vi "AlliGator Phasor Plot Event Registration Refnums.vi"(8 "error in (no error)":errorcluster) -> (0 "error out":errorcluster, 2 "Phasor Plote Display Range Event":refnum<event-registration>, 3 "Phasor Plot Display Event":refnum<event-registration>)   [LabVIEW 2021, in "AlliGator Phasor Plot.lvlib"]
uses:
  AlliGator Phasor Plot.lvlib
panel:
  # "see the License on the block diagram (Ctrl+E or Window:Show Block Diagram)"
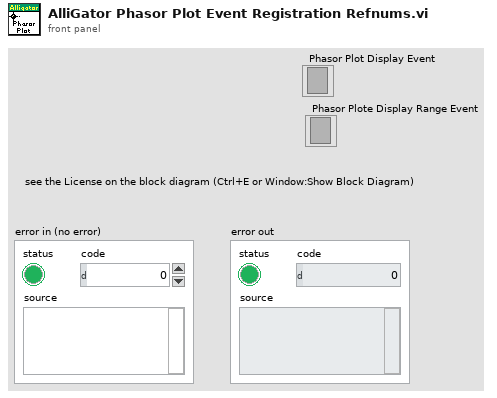
[diagram p1: front panel]
types:
  T1 = typedef "AlliGator Phasor Plot.lvlib/AlliGator Phasor Plot Ctrl Refnums.ctl" = cluster{"Phasor Ratio":refnum<vi>, "Modulus Lifetime":refnum<vi>, "Phasor at cursor (m, phi)":refnum<vi>, "Phase Lifetime":refnum<vi>, "Phasor at cursor (g, s)":refnum<vi>, "Phasor Plor Average Lifetime":refnum<vi>, "Phasor Plot Active":refnum<vi>, "Save Phasor Plot":refnum<vi>, "Image Overlay Color":refnum<vi>, "Phasor Plot Color Scale":refnum<vi>, "Reference 1 Button":refnum<vi>, "Reference 2 Button":refnum<vi>, "True Phasor Plot Value":refnum<vi>, "Phasor Plot Display Range":refnum<vi>, "Phasor Plot Display":refnum<vi>, "Phasor Plot Frequency":refnum<vi>, "Overlay Mode":refnum<vi>}
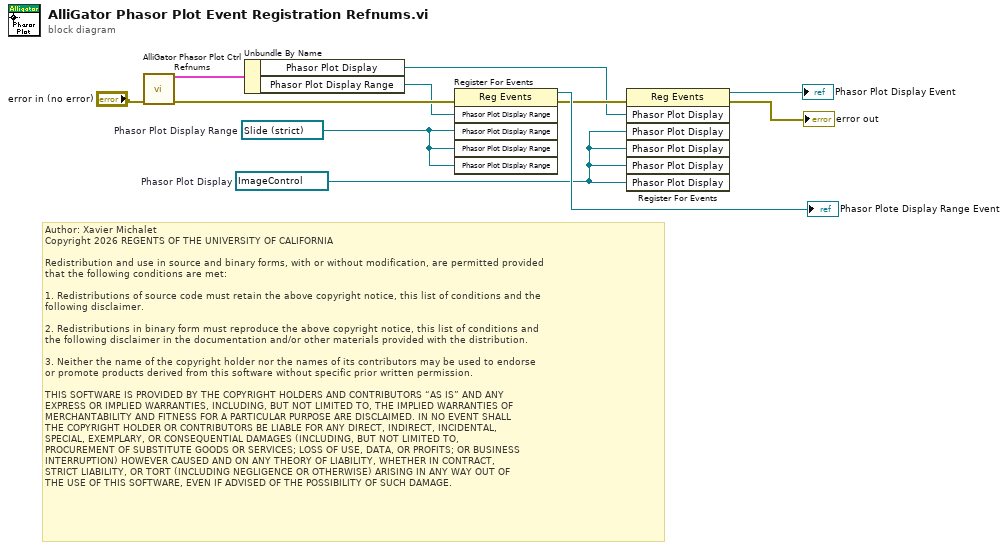
[diagram p0: block diagram]
diagram:
  w10 = refnum<vi> refnum  # Phasor Plot Display Range
  w1 = refnum<vi> refnum  # Phasor Plot Display
  # "Author: Xavier Michalet\nCopyright 2026 REGENTS OF THE UNIVERSITY OF CALIFORNIA\n\nRedistribution and use in source and binary forms, with or without modification, are permitted provided\nthat the following conditions are met:\n\n1. Redistributions of source code must retain the above copyright notice, this list of conditions and the\nfollowing disclaimer.\n\n2. Redistributions in binary form must reproduce the above copyright notice, this list of conditions and\nthe following disclaimer in the documentation and/or other materials provided with the distribution.\n\n3. Neither the name of the copyright holder nor the names of its contributors may be used to endorse \nor promote products derived from this software without specific prior written permission.\n\nTHIS SOFTWARE IS PROVIDED BY THE COPYRIGHT HOLDERS AND CONTRIBUTORS “AS IS” AND ANY \nEXPRESS OR IMPLIED WARRANTIES, INCLUDING, BUT NOT LIMITED TO, THE IMPLIED WARRANTIES OF\nMERCHANTABILITY AND FITNESS FOR A PARTICULAR PURPOSE ARE DISCLAIMED. IN NO EVENT SHALL\nTHE COPYRIGHT HOLDER OR CONTRIBUTORS BE LIABLE FOR ANY DIRECT, INDIRECT, INCIDENTAL, \nSPECIAL, EXEMPLARY, OR CONSEQUENTIAL DAMAGES (INCLUDING, BUT NOT LIMITED TO, \nPROCUREMENT OF SUBSTITUTE GOODS OR SERVICES; LOSS OF USE, DATA, OR PROFITS; OR BUSINESS\nINTERRUPTION) HOWEVER CAUSED AND ON ANY THEORY OF LIABILITY, WHETHER IN CONTRACT, \nSTRICT LIABILITY, OR TORT (INCLUDING NEGLIGENCE OR OTHERWISE) ARISING IN ANY WAY OUT OF\nTHE USE OF THIS SOFTWARE, EVEN IF ADVISED OF THE POSSIBILITY OF SUCH DAMAGE."
  n1 = call "AlliGator Phasor Plot Ctrl Refnums.vi"("error in (no error)"="error in (no error)") -> ("error out"=w8:errorcluster, "Phasor Plot Ctrl Refnums"=w6:T1)  [unwired: 9 in]
  n2 = Unbundle By Name(w6) -> ("Phasor Plot Display"=w4:refnum<vi>, "Phasor Plot Display Range"=w5:refnum<vi>)
  n3 = register-events(error in=w8, w5, w10, w10, w10) -> (reference out=→"Phasor Plote Display Range Event":refnum<event-registration>, error out=w9:errorcluster)  [unwired: 1 in]
  n4 = register-events(error in=w9, w4, w1, w1, w1, w1) -> (reference out=→"Phasor Plot Display Event":refnum<event-registration>, error out=→"error out":errorcluster)  [unwired: 1 in]
